vi "OwnOop20261013_CreateOverride.vi"() -> ()   [LabVIEW 2024]
uses:
  <resource>/Framework/Providers/LVClassLibrary/NewAccessors/MemberVICreation.lvlib
panel:
  out "error out":errorcluster caption="错误输出"
  in  "Save Class Path":path
  in  "Member Path":path
  in  "Memory Name":string
  in  "Child Class Path":path
  in  "Parent Method Path":path
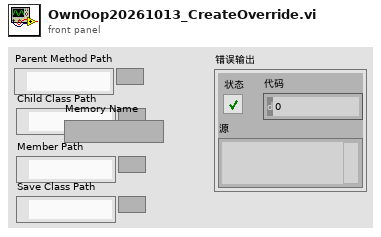
[diagram p1: front panel]
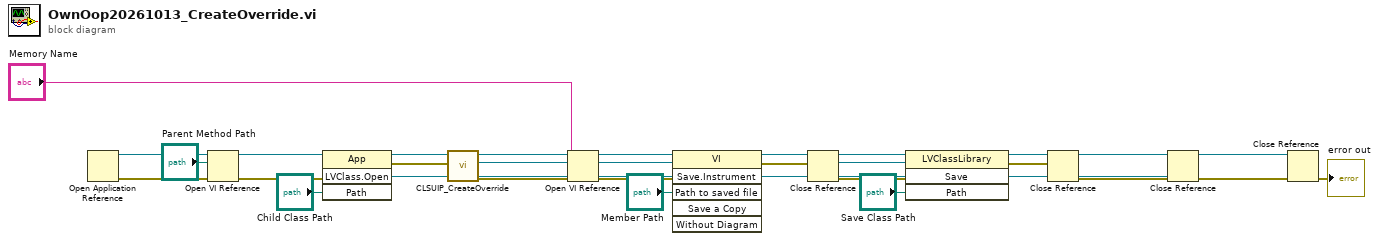
[diagram p0: block diagram]
diagram:
  n1 = Open Application Reference() -> (0:w19:errorcluster, 3:w20:refnum<vi>)  [unwired: 4 in]
  n2 = Open VI Reference(application reference (local)=w20, vi path="Parent Method Path", error in (no error)=w19) -> (vi reference=w16:refnum<vi>, error out=w17:errorcluster)  [unwired: 3 in]
  n3 = invoke class="App" method="LVClass.Open"(reference=w20, error in=w17, "Path"="Child Class Path") -> (error out=w14:errorcluster, "LVClass.Open"=w15:refnum<vi>)  [unwired: 1 in, 2 out]
  n4 = call <resource>:"CLSUIP_CreateOverride.vi"("error in (no error)"=w14, "Child class"=w15, "Parent Method"=w16) -> ("error out"=w12:errorcluster, "Child class out"=w7:refnum<vi>)  [unwired: 5 in, 2 out]
  n5 = Open VI Reference(application reference (local)=w20, vi path="Memory Name", error in (no error)=w12) -> (vi reference=w11:refnum<vi>, error out=w9:errorcluster)  [unwired: 3 in]
  n6 = invoke class="VI" method="Save.Instrument"(reference=w11, error in=w9, "Path to saved file"="Member Path") -> (error out=w8:errorcluster)  [unwired: 3 in, 5 out]
  n7 = Close Reference(reference=w11, error in (no error)=w8) -> (error out=w5:errorcluster)
  n8 = invoke class="LVClassLibrary" method="Save"(reference=w7, error in=w5, "Path"="Save Class Path") -> (error out=w4:errorcluster)  [unwired: 1 in, 3 out]
  n9 = Close Reference(reference=w16, error in (no error)=w4) -> (error out=w3:errorcluster)
  n10 = Close Reference(reference=w15, error in (no error)=w3) -> (error out=w2:errorcluster)
  n11 = Close Reference(reference=w20, error in (no error)=w2) -> (error out=→"error out":errorcluster)
